vi "Double It.vi"(0 "x":i32=3) -> (1 "Doubled":i32)   [LabVIEW 2026]
doc: "Round21 nested-chain grandchild (deepest layer of the three-level Call chain): doubles an int32. Panel: x in (conIdx0, required), Doubled out (conIdx1, recommended). Called by Sum Of Doubles.vi, which is called by Nested Chain Demo.vi."
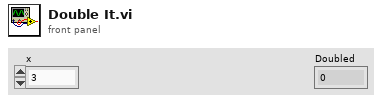
[diagram p1: front panel]
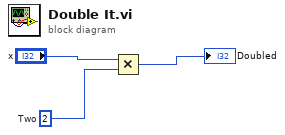
[diagram p0: block diagram]
diagram:
  w2 = 2  # Two
  n1 = Multiply(x="x", y=w2) -> (x*y=→"Doubled":i32)
